vi "lvmcp_eventsel.vi"() -> ()   [LabVIEW 2026]
panel:
  out "error out":errorcluster
  out "selectors":string[](array[string])
  in  "reference":refnum<vi>
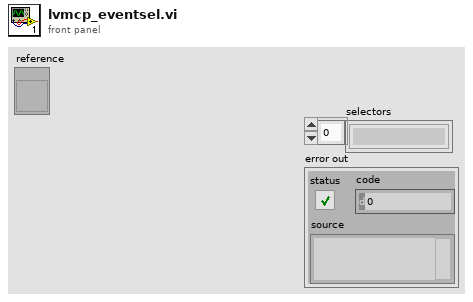
[diagram p1: front panel]
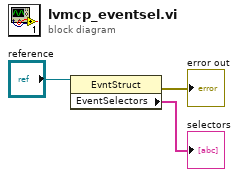
[diagram p0: block diagram]
diagram:
  n1 = property class="EvntStruct"(reference="reference") -> (error out=→"error out":errorcluster, "EventSelectors"=→"selectors":string[])  [unwired: 1 in, 1 out]
